vi "libssh2_session_banner_get.vi"(8 "error in (no error)":errorcluster, 11 "session":T1) -> (0 "error out":errorcluster, 2 "banner":string)   [LabVIEW 2017, in "libssh2.lvlib"]
doc: "Get the banner that was sent by the server when a session was established."
uses:
  libssh2.lvlib
  Session Refnum.ctl
  Not A Session.vi
  <vilib>/Utility/error.llb/Error Cluster From Error Code.vi
  Global Settings.vi
  Read Session Refnum.vi
  <vilib>/Utility/semaphor.llb/Acquire Semaphore.vi
  <vilib>/Utility/semaphor.llb/Release Semaphore.vi
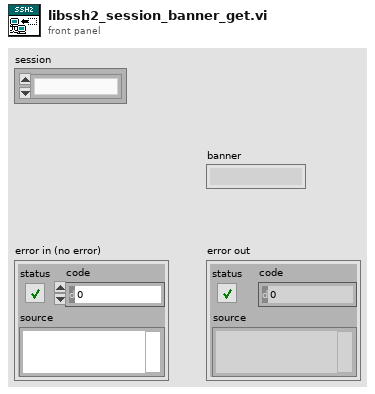
[diagram p1: front panel]
types:
  T1 = typedef "libssh2.lvlib/Session Refnum.ctl" = refnum<k1>
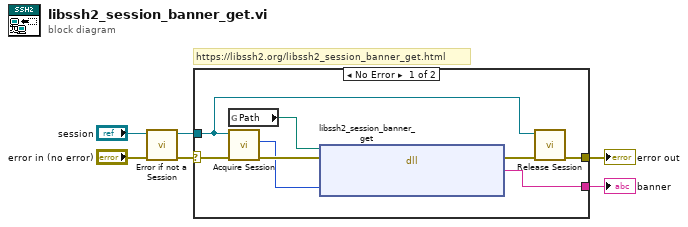
[diagram p0: block diagram]
diagram:
  # "https://libssh2.org/libssh2_session_banner_get.html"
  n1 = call "Error if not a Session.vi"("error in (no error)"="error in (no error)", "session"="session") -> ("error out"=w4:errorcluster, "session out"=w2:T1)  [unwired: 8 in]
  n2 = case shown="No Error" w4 {
    selector: w4 -> [w7 w15]
    tunnel: [w9 w15] -> w6
    tunnel: w2 -> [w8 _]
    tunnel: [w10 _] -> w1
    frame No Error {
      n3 = global read "Global Settings.vi" "Path"() -> (w11:path)
      n4 = call "Acquire Session.vi"("error in (no error)"=w7, "session"=w8) -> ("error out"=w13:errorcluster, "LIBSSH2_SESSION*"=w12:u64)  [unwired: 7 in, 1 out]
      n5 = dll-call lib="?" fn="libssh2_session_banner_get"(path in=w11, error in=w13, "session"=w12) -> (error out=w14:errorcluster, "return value"=w10:string)  [unwired: 2 in, 1 out]
      n6 = call "Release Session.vi"("error in (no error)"=w14, "session"=w8) -> ("error out"=w9:errorcluster)  [unwired: 9 in]
    }
    frame Error {
    }
  }
  "error out" <- w6
  "banner" <- w1
